vi "Relative Path Constant.vi"(11 "error in":errorcluster) -> (4 "path text":string, 15 "error out":errorcluster)   [LabVIEW 2024]
doc: "Fixture containing one relative path constant."
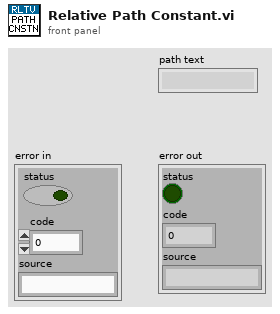
[diagram p1: front panel]
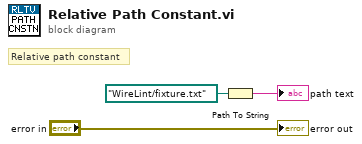
[diagram p0: block diagram]
diagram:
  # "Relative path constant"
  n1 = Path To String(path=path "WireLint/fixture.txt" ("relative path")) -> (string=→"path text":string)
  "error out" <- "error in"
